vi "Test U8 Subscriber.vi"() -> ()   [LabVIEW 2021]
uses:
  ChannelCommon/typedef/Direction.ctl
  CIF_Iceoryx_PCAP_Universal.lvclass
  ChannelCommon/typedef/New FIFO Instance Response.ctl
  Iceorxy Utilities/Typedef/PCAP Config.ctl
  ChannelCommon/typedef/New FIFO Config.ctl
  ChannelCommon/typedef/FIFO Flags.ctl
  Iceorxy Utilities/Typedef/PCAP Linktype.ctl
  ChannelCommon/ChannelCommon.lvlib
  Iceorxy Utilities/Iceoryx Channel Utilities.lvlib
panel:
  in  "millisecond multiple":u32
  out "U8 Data":u8[](array[numeric])
  in  "stop":bool
  out "timed out?":bool
  out "error out":errorcluster
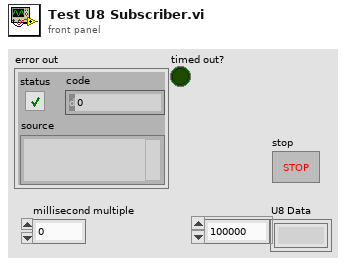
[diagram p1: front panel]
types:
  T1 = typedef "Iceoryx Channel Utilities.lvlib/PCAP Config.ctl" = cluster{"New FIFO Config":T2, "Linktype":T4, "Linktype Override":u32, "Type Name Override":string}
  T2 = typedef "ChannelCommon.lvlib/New FIFO Config.ctl" = cluster{"Max Bytes/Msg":u64, "Max Msg/FIFO":u64, "FIFO Flags":T3, "Best Effort Subscribers":u32, "Backpressure Subscribers":u32}
  T3 = typedef "ChannelCommon.lvlib/FIFO Flags.ctl" = cluster{"Backpressure":bool, "Extended Config":bool}
  T4 = typedef "Iceoryx Channel Utilities.lvlib/PCAP Linktype.ctl" = u32
  T5 = typedef "ChannelCommon.lvlib/New FIFO Instance Response.ctl" = cluster{"Publisher":string, "Custom Data":u8[]}
  T6 = typedef "ChannelCommon.lvlib/Direction.ctl" = enum8{"Publisher", "Subscriber"}
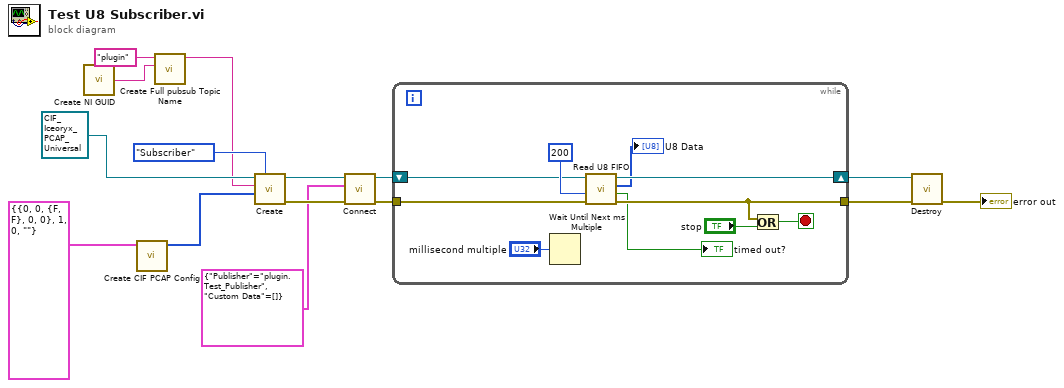
[diagram p0: block diagram]
diagram:
  n1 = call <vilib>:"Create NI GUID.vi"() -> ("NI GUID"=w2:string)
  n2 = call "Create CIF PCAP Config.vi"("PCAP FIFO Config"=T1 {"New FIFO Config"={"Max Bytes/Msg"=0, "Max Msg/FIFO"=0, "FIFO Flags"={"Backpressure"=FALSE, "Extended Config"=FALSE}, "Best Effort Subscribers"=0, "Backpressure Subscribers"=0}, "Linktype"=1, "Linktype Override"=0, "Type Name Override"=""}) -> ("Flattened PCAP FIFO Config"=w4:u8[])  [unwired: 10 in]
  n3 = call "Create Full pubsub Topic Name.vi"("Topic"=w2, "Plugin name"="plugin") -> ("Full Topic"=w1:string)  [unwired: 8 in, 1 out]
  n4 = call-dynamic "Create.vi"("Direction"=Direction."Subscriber", "Custom Config Data"=w4, "Name"=w1, "CIFFIFO in"=refnum<class "CIF_Iceoryx_PCAP_Universal.lvclass"> refnum ("CIF_CIPC_Fifo_U8.lvclass")) -> ("error out"=w12:errorcluster, "CIFFIFO out"=w13:refnum<class "CIF_Iceoryx_PCAP_Universal.lvclass">)  [unwired: 6 in]
  n5 = call-dynamic "Connect.vi"("error in (no error)"=w12, "Connection"=T5 {"Publisher"="plugin.Test_Publisher", "Custom Data"=[]}, "CIF_Iceoryx_PCAP"=w13) -> ("error out"=w9:errorcluster, "CIF_Iceoryx_PCAP"=w11:refnum<class "CIF_Iceoryx_PCAP_Universal.lvclass">)  [unwired: 7 in]
  n6 = while {
    shift-right: [w25] -> w15
    shift-left: w11 -> [w23]
    tunnel: w9 -> [w22]
    tunnel: [w19] -> w8
    stop <- w17 stop-if-true
    n7 = Wait Until Next ms Multiple(millisecond multiple="millisecond multiple") -> ()  [unwired: 1 out]
    n8 = call-dynamic "Read U8 FIFO.vi"("error in (no error)"=w22, "Timeout (ms)"=200, "CIFFIFO in"=w23) -> ("error out"=w19:errorcluster, "timed out?"=→"timed out?":bool, "Data out"=→"U8 Data":u8[], "CIFFIFO out"=w25:refnum<class "CIF_Iceoryx_PCAP_Universal.lvclass">)  [unwired: 4 in, 1 out]
    n9 = Or(x=w19, y="stop") -> (x .or. y?=w17:bool)
  }
  n10 = call-dynamic "Destroy.vi"("error in (no error)"=w8, "Icoryx_PCAP in"=w15) -> ("error out"=→"error out":errorcluster)  [unwired: 8 in, 1 out]
